vi "Main.vi"() -> ()   [LabVIEW 2020]
doc: "This template is for the Queued Message Handler design pattern.\n\nThe Event Handling Loop generates messages based on user interface actions.\n\nThe Message Handling Loop processes messages generated by the Event Handling Loop, or by other messages. The messages are string values, so new messages can be added easily to the Message Cases case structure in the Message Handling Loop. Each message cluster can also provide an optional value for Message Data, which is a variant that can be converted to whatever message-specific data is required."
uses:
  <vilib>/ErrorRing/Error Ring.xnode
  controls/oled UI Data.ctl
  support/Message Queue/oled Message Queue.lvlib
  support/User Event - Stop/oled User Event - Stop.lvlib
  support/Message Queue/Enqueue Message (Single).vi
  controls/HL Acq Data.ctl
  <vilib>/DAQmx/read.llb/DAQmx Read (Analog DBL 1Chan 1Samp).vi
  <vilib>/Instr/_visa.llb/VISA Configure Serial Port (Instr).vi
  <vilib>/DAQmx/create/channels.llb/DAQmx Create Channel (AI-Voltage-Basic).vi
  support/Message Queue/Enqueue Message (Array).vi
  controls/Acquisition data --typedef.ctl
  controls/Graph data --typedef.ctl
  <vilib>/Utility/error.llb/Error Cluster From Error Code.vi
  controls/Color --typedef.ctl
panel:
  in  "Color":T1 caption="Color de emisión"
  in  "Inicio de Barrido (V)":dbl
  out "Status":string
  in  "milliseconds to wait":i32=200
  out "Eff L-V":cluster{dbl[], dbl[]}(graph) caption="L-V"
  out "EFf I-V":cluster{dbl[], dbl[]}(graph) caption="L-V"
  in  "Puerto serial Fuente":refnum<visa-resource-name>="COM1"
  out "J-V":cluster{dbl[], dbl[]}(graph)
  out "L-V":cluster{dbl[], dbl[]}(graph)
  in  "OLED A":dbl=0.7 caption="Area del OLED [cm2]"
  in  "OLED-PD dist":dbl=1.0 caption="Distancia OLED-fotodiodo [cm]"
  in  "Protection C":dbl=0.1 caption="Corriente de Proteccion [A]\n(0.1-0.3A recomendado)"
  in  "Max V":dbl=10.0 caption="Voltaje máximo [V]\n(20V max. recomendado)"
  in  "Iniciar":bool
  in  "Step #":dbl=100.0 caption="Numero de pasos\n(100-250 recomendado)"
  in  "Exit":bool
  # "Sistema de caracterización de OLEDs"
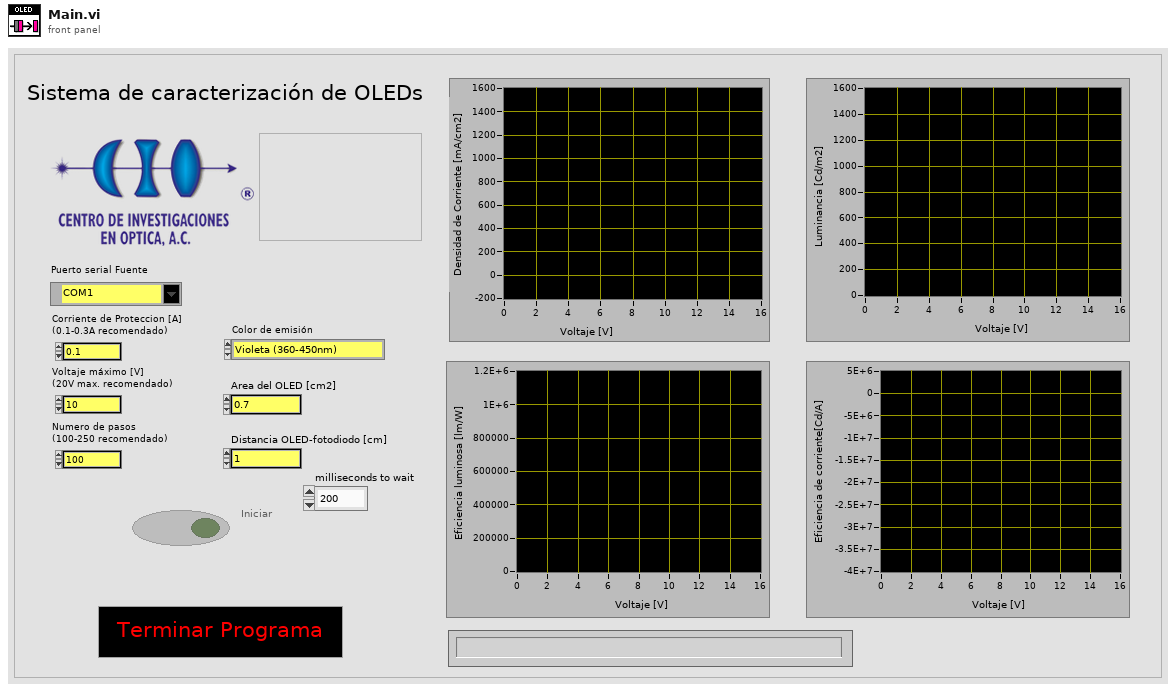
[diagram p1: front panel]
types:
  T1 = typedef "Color --typedef.ctl" = enum16{"Violeta (360-450nm)", "Azul (450-500nm)", "Verde(500-570nm)", "Amarillo (570-590nm)", "Naranja (600-610nm)", "Rojo (610-670nm)", "Blanco"}
  T2 = typedef "oled UI Data.ctl" = cluster{"Status":string, "Puerto serial":refnum<visa-resource-name>, "AI task":refnum<k21>, "Protection C":dbl, "Sweep start V":dbl, "Max V":dbl, "delta V":dbl, "Graph data":T3}
  T3 = typedef "Graph data --typedef.ctl" = cluster{"Voltaje [V]":dbl[], "Corriente [mA]":dbl[], "Densidad de corriente [CD/A]":dbl[], "Iluminancia [Lm/m2]":dbl[], "Luminance [Cd/m2]":dbl[], "Ef corriente [Cd/A]":dbl[], "Ef Luminosa [Cd/W]":dbl[], "V detector [V]":dbl[], "Pin [W]":dbl[]}
  T4 = cluster{"User event - Stop":refnum<user-event>, "User event - Sleep HL":refnum<user-event>, "User event -  Wake HL":refnum<user-event>}
  T5 = typedef "oled Message Queue.lvlib/All Message Queues.ctl" = cluster{"UI":refnum<queue>}
  T6 = enum8{"Enabled", "Disabled", "Disabled and Grayed Out"}
  T7 = typedef "HL Acq Data.ctl" = cluster{"dV":dbl, "Vmax":dbl, "Vo":dbl}
  T8 = typedef "Acquisition data --typedef.ctl" = cluster{"Iluminancia  lm/m2":dbl, "DAQ AV":dbl, "Luminancia (Cd/m2)":dbl, "Pin(W)":dbl, "SM V":dbl, "SM I":dbl, "OLED Area cm2":dbl}
  T9 = cluster{"Voltaje [V]":dbl[], "Luminance [Cd/m2]":dbl[]}
  T10 = cluster{"Voltaje [V]":dbl[], "V detector [V]":dbl[]}
  T11 = cluster{"Voltaje [V]":dbl[], "Ef corriente [Cd/A]":dbl[]}
  T12 = cluster{"Voltaje [V]":dbl[], "Corriente [mA]":dbl[]}
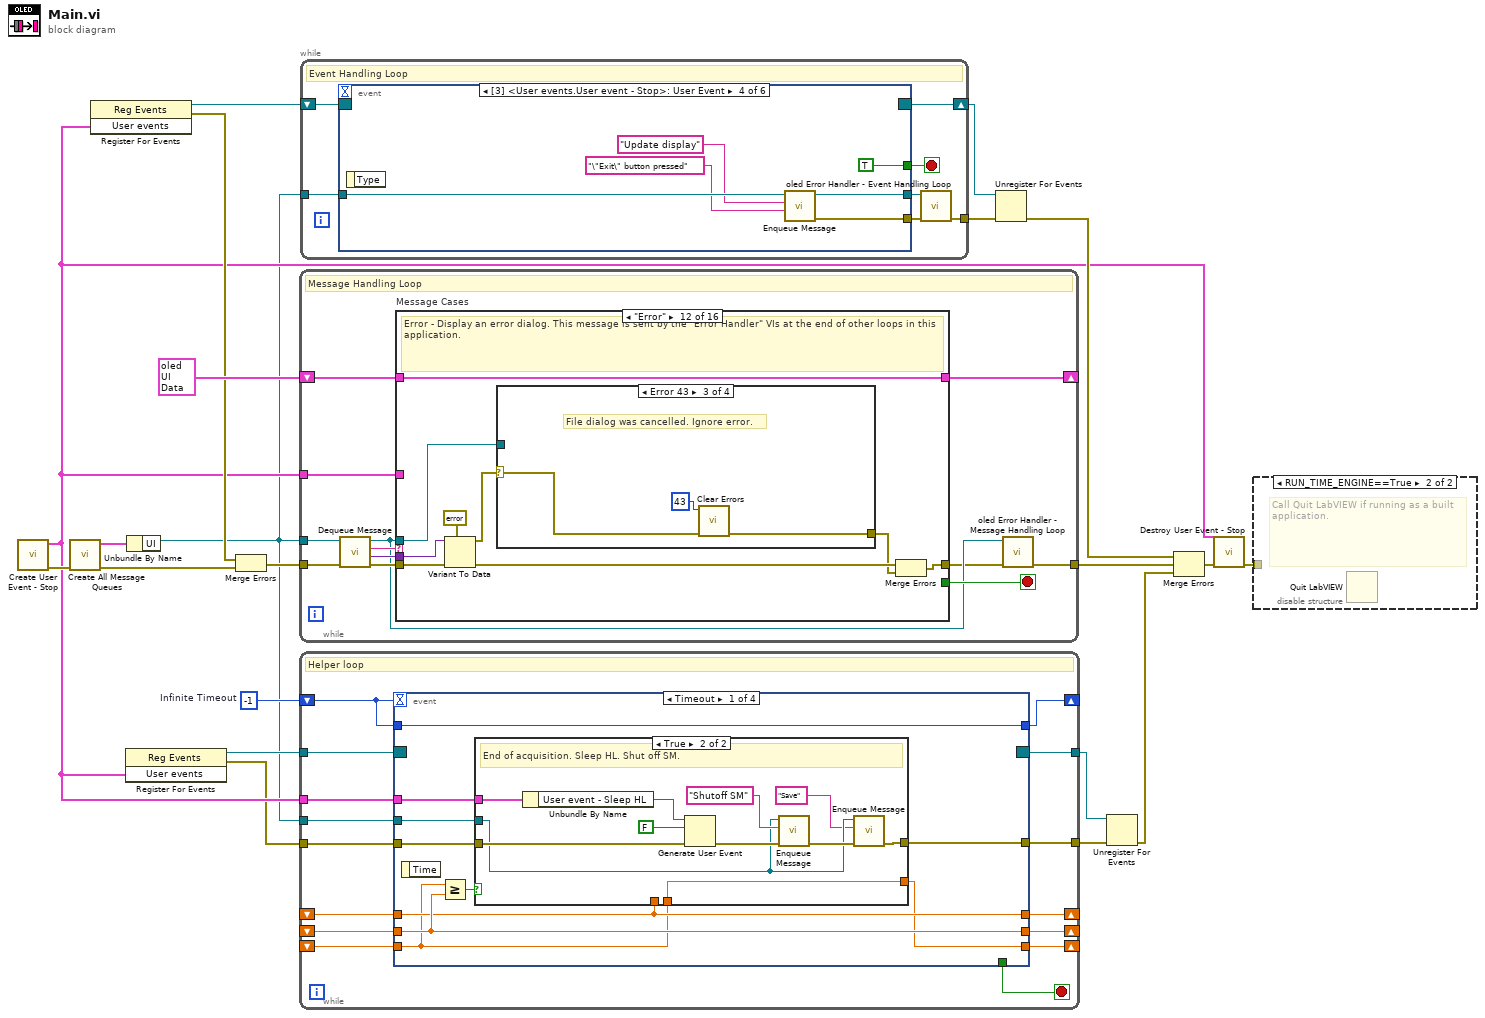
[diagram p0: block diagram]
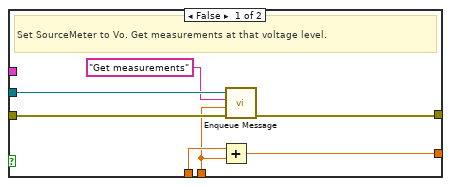
[diagram p2: hidden frame]
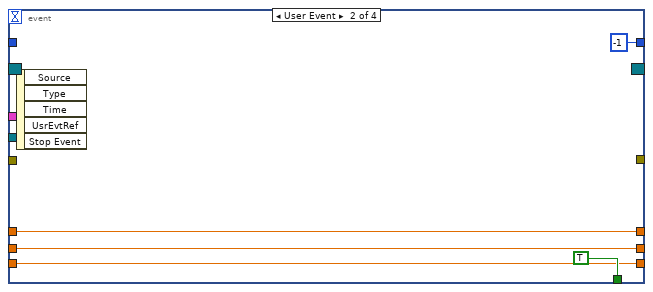
[diagram p3: hidden frame]
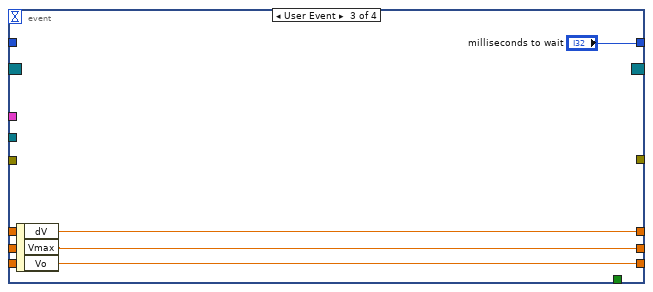
[diagram p4: hidden frame]
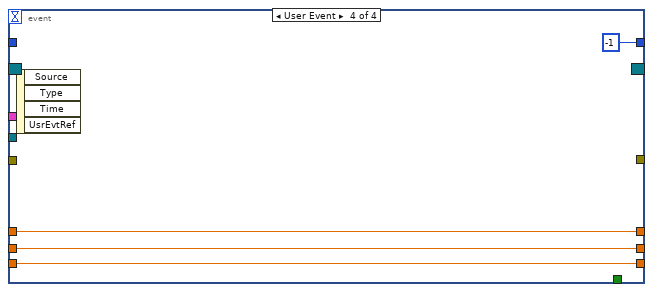
[diagram p5: hidden frame]
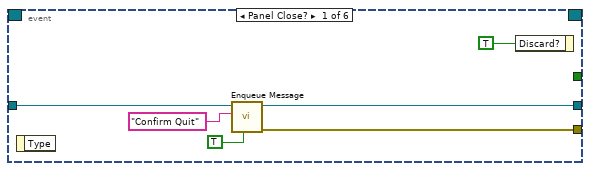
[diagram p6: hidden frame]
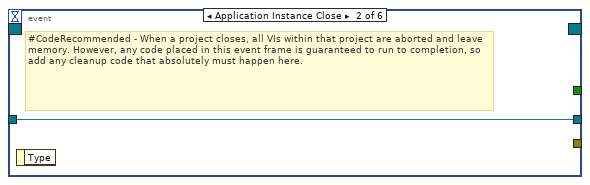
[diagram p7: hidden frame]
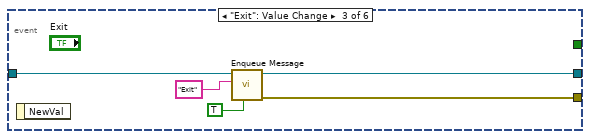
[diagram p8: hidden frame]
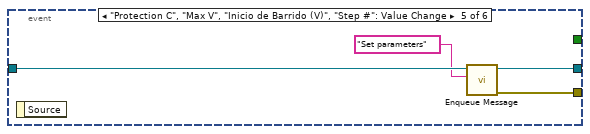
[diagram p9: hidden frame]
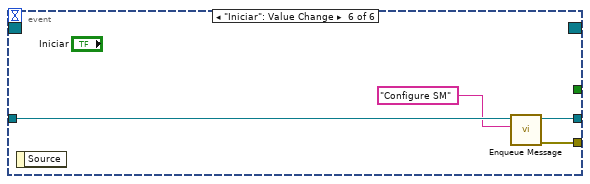
[diagram p10: hidden frame]
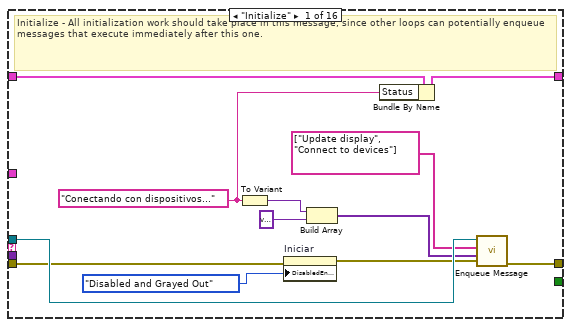
[diagram p11: hidden frame]
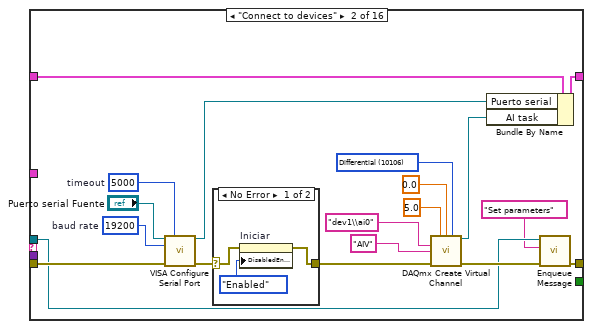
[diagram p12: hidden frame]
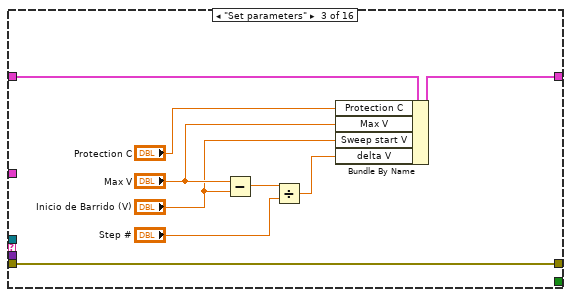
[diagram p14: hidden frame]
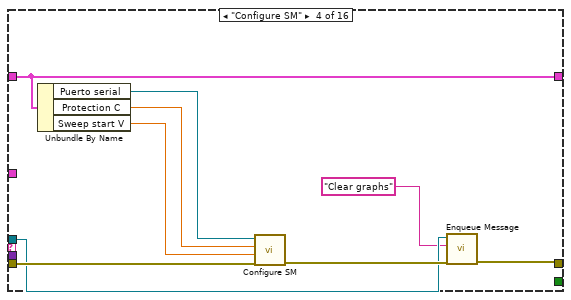
[diagram p15: hidden frame]
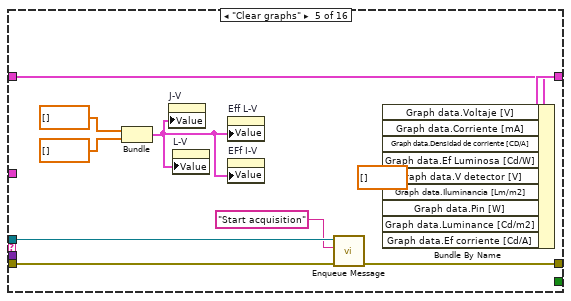
[diagram p16: hidden frame]
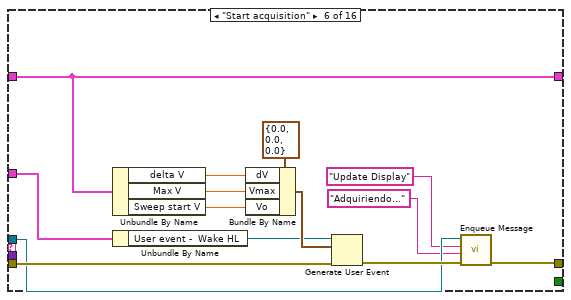
[diagram p17: hidden frame]
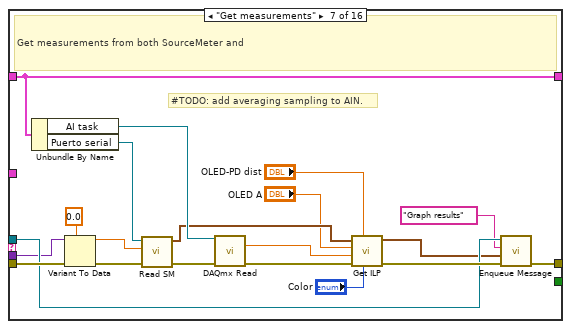
[diagram p18: hidden frame]
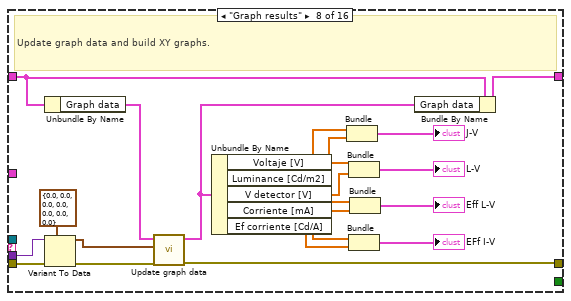
[diagram p19: hidden frame]
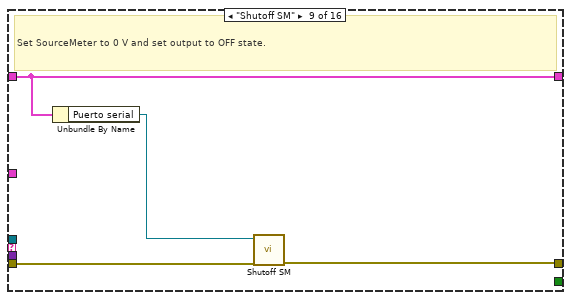
[diagram p20: hidden frame]
diagram:
  w9 = -1  # Infinite Timeout
  n1 = call "Create User Event - Stop.vi"() -> ("error out"=w19:errorcluster, "User events"=w4:T4)  [unwired: 10 in]
  n2 = call "Create All Message Queues.vi"("error in (no error)"=w19) -> ("error out"=w21:errorcluster, "Message Queues out"=w20:T5)  [unwired: 9 in]
  n3 = register-events(w4) -> (reference out=w12:refnum<event-registration>, error out=w10:errorcluster)  [unwired: 2 in]
  n4 = register-events(w4) -> (reference out=w8:refnum<event-registration>, error out=w2:errorcluster)  [unwired: 2 in]
  n5 = Unbundle By Name(w20) -> ("UI"=w1:refnum<queue>)
  n6 = Merge Errors(w10, w21) -> (w11:errorcluster)
  n7 = while {
    tunnel: w1 -> [w25]
    shift-right: [w32] -> _
    shift-left: T2 {"Status"="", "Puerto serial"="", "AI task"="", "Protection C"=0.0, "Sweep start V"=0.0, "Max V"=0.0, "delta V"=0.0, "Graph data"={"Voltaje [V]"=[], "Corriente [mA]"=[], "Densidad de corriente [CD/A]"=[], "Iluminancia [Lm/m2]"=[], "Luminance [Cd/m2]"=[], "Ef corriente [Cd/A]"=[], "Ef Luminosa [Cd/W]"=[], "V detector [V]"=[], "Pin [W]"=[]}} ("Data Cluster") -> [w33]
    tunnel: w4 -> [w30]
    tunnel: w11 -> [w29]
    tunnel: [w23] -> w6
    stop <- w31 stop-if-true
    # "Message Handling Loop"
    n8 = call "Dequeue Message.vi"("error in (no error)"=w29, "Message Queue"=w25) -> ("error out"=w28:errorcluster, "Message Data"=w26:variant, "Message"=w27:string, "dup Message Queue"=w24:refnum<queue>)  [unwired: 6 in]
    n9 = case "Message Cases" shown="\"Error\"" w27 {
      selector: w27 -> [_ _ _ _ _ _ _ _ _ _ _ _ _ _ _ w227]
      tunnel: w24 -> [w42 w49 _ w79 w88 w99 w122 _ _ _ _ w171 w196 _ w226 _]
      tunnel: w28 -> [w35 w64 w77 w82 w90 w105 w130 w149 w153 w155 w169 w179 w200 w203 w220 _]
      tunnel: [w45 w50 w77 w80 w89 w100 w123 w141 w152 w154 w170 w174 w198 w201 w223 w228] -> w22
      tunnel: w33 -> [w44 w60 w75 w86 w91 w103 w129 w144 w151 w157 w160 w178 w199 w202 w216 w229]
      tunnel: [w43 w58 w70 w86 w93 w103 w129 w143 w151 w157 w158 w178 w199 w202 w216 w229] -> w32
      tunnel: [_ _ _ _ _ _ _ _ _ _ _ _ _ _ TRUE _] -> w31
      tunnel: w26 -> [_ _ _ _ _ _ w113 w147 _ _ w168 w177 _ _ w217 _]
      tunnel: w30 -> [_ _ _ _ _ w106 _ _ _ _ _ _ _ _ w222 _]
      frame "Initialize" {
        w37 = "Conectando con dispositivos..." ("Initial Message")
        # "Initialize - All initialization work should take place in this message, since other loops can potentially enqueue messages that execute immediately after this one."
        n10 = To Variant(anything=w37) -> (Variant=w40:variant)
        n11 = property on="Iniciar" class="Bool (strict)"(error in=w35, "DisabledEnum"=T6."Disabled and Grayed Out" ("Disabled")) -> (error out=w34:errorcluster)  [unwired: 1 in, 1 out]
        n12 = Build Array(w40, variant ("element")) -> (w38:variant[])
        n13 = Bundle By Name(cluster=w44, "Status"=w37) -> (w43:T2)
        n14 = call-poly "Enqueue Message.vi"("error in (no error)"=w34, "Message Data Array"=w38, "Message Array"=string[] ["Update display", "Connect to devices"] ("Message"), "Message Queue"=w42) -> ("error out"=w45:errorcluster)  [unwired: 6 in, 1 out]
      }
      frame "Connect to devices" {
        w53 = 10106 items=["Default"=-1, "RSE"=10083, "NRSE"=10078, "Differential"=10106, "Pseudodifferential"=12529] ("input terminal configuration")
        w61 = u32 5000  # timeout
        w62 = u32 19200  # baud rate
        n15 = call-poly "VISA Configure Serial Port"("VISA resource name"="Puerto serial Fuente", "timeout (10sec)"=w61, "baud rate (9600)"=w62, "error in (no error)"=w64) -> ("VISA resource name out"=w59:refnum<visa-resource-name>, "error out"=w47:errorcluster)  [unwired: 3 in, 7 out]
        n16 = case shown="No Error" w47 {
          selector: w47 -> [w67 w68]
          tunnel: [w66 w68] -> w46
          frame No Error {
            n17 = property on="Iniciar" class="Bool (strict)"(error in=w67, "DisabledEnum"=T6."Enabled" ("Disabled")) -> (error out=w66:errorcluster)  [unwired: 1 in, 1 out]
          }
          frame Error {
          }
        }
        n18 = call-poly <vilib>:"DAQmx Create Virtual Channel.vi"("maximum value"=5.0, "minimum value"=0.0, "input terminal configuration"=w53, "physical channels"="dev1\\ai0", "name to assign"="AIV", "error in"=w46) -> ("task out"=w52:refnum<k21>, "error out"=w51:errorcluster)  [unwired: 8 in]
        n19 = Bundle By Name(cluster=w60, "Puerto serial"=w59, "AI task"=w52) -> (w58:T2)
        n20 = call-poly "Enqueue Message.vi"("error in (no error)"=w51, "Message"="Set parameters", "Message Queue"=w49) -> ("error out"=w50:errorcluster)  [unwired: 7 in, 1 out]
      }
      frame "Set parameters" {
        n21 = Subtract(x="Max V", y="Inicio de Barrido (V)") -> (x-y=w76:dbl)
        n22 = Divide(x=w76, y="Step #") -> (x/y=w71:dbl)
        n23 = Bundle By Name(cluster=w75, "Protection C"="Protection C", "Max V"="Max V", "Sweep start V"="Inicio de Barrido (V)", "delta V"=w71) -> (w70:T2)
      }
      frame "Configure SM" {
        n24 = Unbundle By Name(w86) -> ("Puerto serial"=w84:refnum<visa-resource-name>, "Protection C"=w83:dbl, "Sweep start V"=w85:dbl)
        n25 = call "Configure SM.vi"("error in (no error)"=w82, "Sweep start V"=w85, "Protection C"=w83, "Puerto serial"=w84) -> ("error out"=w81:errorcluster)  [unwired: 7 in]
        n26 = call-poly "Enqueue Message.vi"("error in (no error)"=w81, "Message"="Clear graphs", "Message Queue"=w79) -> ("error out"=w80:errorcluster)  [unwired: 7 in, 1 out]
      }
      frame "Clear graphs" {
        w92 = dbl[] []
        n27 = Bundle(dbl[] [], dbl[] []) -> (w94:cluster{dbl[], dbl[]})  [unwired: 1 out]
        n28 = property on="J-V" class="XYGraph (strict)"("Value"=w94) -> ()  [unwired: 2 in, 2 out]
        n29 = property on="L-V" class="XYGraph (strict)"("Value"=w94) -> ()  [unwired: 2 in, 2 out]
        n30 = property on="Eff L-V" class="XYGraph (strict)"("Value"=w94) -> ()  [unwired: 2 in, 2 out]
        n31 = property on="EFf I-V" class="XYGraph (strict)"("Value"=w94) -> ()  [unwired: 2 in, 2 out]
        n32 = call-poly "Enqueue Message.vi"("error in (no error)"=w90, "Message"="Start acquisition", "Message Queue"=w88) -> ("error out"=w89:errorcluster)  [unwired: 7 in, 1 out]
        n33 = Bundle By Name(cluster=w91, "Graph data.Voltaje [V]"=w92, "Graph data.Corriente [mA]"=w92, "Graph data.Densidad de corriente [CD/A]"=w92, "Graph data.Ef Luminosa [Cd/W]"=w92, "Graph data.V detector [V]"=w92, "Graph data.Iluminancia [Lm/m2]"=w92, "Graph data.Pin [W]"=w92, "Graph data.Luminance [Cd/m2]"=w92, "Graph data.Ef corriente [Cd/A]"=w92) -> (w93:T2)
      }
      frame "Start acquisition" {
        n34 = Unbundle By Name(w103) -> ("delta V"=w102:dbl, "Max V"=w108:dbl, "Sweep start V"=w107:dbl)
        n35 = Unbundle By Name(w106) -> ("User event -  Wake HL"=w104:refnum<user-event>)
        n36 = Bundle By Name(cluster=T7 {"dV"=0.0, "Vmax"=0.0, "Vo"=0.0} ("event data"), "dV"=w102, "Vmax"=w108, "Vo"=w107) -> (w109:T7)
        n37 = Generate User Event(user event=w104, event data cluster=w109, error in=w105) -> (error out=w101:errorcluster)  [unwired: 1 in, 1 out]
        n38 = call-poly "Enqueue Message.vi"("error in (no error)"=w101, "Message Data"="Adquiriendo..." ("Message"), "Message"="Update Display", "Message Queue"=w99) -> ("error out"=w100:errorcluster)  [unwired: 6 in, 1 out]
      }
      frame "Get measurements" {
        # "#TODO: add averaging sampling to AIN."
        # "Get measurements from both SourceMeter and"
        n39 = Unbundle By Name(w129) -> ("AI task"=w126:refnum<k21>, "Puerto serial"=w128:refnum<visa-resource-name>)
        n40 = Variant To Data(error in=w130, type=0.0, Variant=w113) -> (data=w112:dbl, error out=w115:errorcluster)
        n41 = call "Read SM.vi"("error in (no error)"=w115, "Vo"=w112, "Puerto serial"=w128) -> ("error out"=w127:errorcluster, "Acquistion Data"=w119:T8)  [unwired: 7 in]
        n42 = call-poly <vilib>:"DAQmx Read.vi"("task/channels in"=w126, "error in"=w127) -> ("data"=w118:dbl, "error out"=w125:errorcluster)  [unwired: 11 in, 1 out]
        n43 = call "Get ILP.vi"("Color"="Color", "OLED-PD dist"="OLED-PD dist", "error in (no error)"=w125, "DAQ V"=w118, "OLED A"="OLED A", "Acquistion Data"=w119) -> ("error out"=w124:errorcluster, "Acquistion Data"=w120:T8)  [unwired: 4 in]
        n44 = call-poly "Enqueue Message.vi"("error in (no error)"=w124, "Message Data"=w120, "Message"="Graph results", "Message Queue"=w122) -> ("error out"=w123:errorcluster)  [unwired: 6 in, 1 out]
      }
      frame "Graph results" {
        # "Update graph data and build XY graphs."
        n45 = Unbundle By Name(w144) -> ("Graph data"=w145:T3)
        n46 = Variant To Data(error in=w149, type=T8 {"Iluminancia  lm/m2"=0.0, "DAQ AV"=0.0, "Luminancia (Cd/m2)"=0.0, "Pin(W)"=0.0, "SM V"=0.0, "SM I"=0.0, "OLED Area cm2"=0.0} ("output cluster"), Variant=w147) -> (data=w146:T8, error out=w142:errorcluster)
        n47 = call "Update graph data.vi"("error in (no error)"=w142, "Acquisition data"=w146, "Graph data"=w145) -> ("error out"=w141:errorcluster, "Graph data"=w135:T3)  [unwired: 7 in]
        n48 = Unbundle By Name(w135) -> ("Voltaje [V]"=w134:dbl[], "Luminance [Cd/m2]"=w140:dbl[], "V detector [V]"=w133:dbl[], "Corriente [mA]"=w132:dbl[], "Ef corriente [Cd/A]"=w131:dbl[])
        n49 = Bundle("Voltaje [V]"=w134, "Luminance [Cd/m2]"=w140) -> (→"J-V":T9)  [unwired: 1 in]
        n50 = Bundle("Voltaje [V]"=w134, "V detector [V]"=w133) -> (→"L-V":T10)  [unwired: 1 in]
        n51 = Bundle("Voltaje [V]"=w134, "Ef corriente [Cd/A]"=w131) -> (→"EFf I-V":T11)  [unwired: 1 in]
        n52 = Bundle("Voltaje [V]"=w134, "Corriente [mA]"=w132) -> (→"Eff L-V":T12)  [unwired: 1 in]
        n53 = Bundle By Name(cluster=w144, "Graph data"=w135) -> (w143:T2)
      }
      frame "Shutoff SM" {
        # "Set SourceMeter to 0 V and set output to OFF state."
        n54 = Unbundle By Name(w151) -> ("Puerto serial"=w150:refnum<visa-resource-name>)
        n55 = call "Shutoff SM.vi"("error in (no error)"=w153, "Puerto serial"=w150) -> ("error out"=w152:errorcluster)  [unwired: 8 in, 1 out]
      }
      frame "Save" {
        n56 = Unbundle By Name(w157) -> ("Graph data"=w156:T3)
        n57 = call "Write file.vi"("error in (no error)"=w155, "Graph data"=w156) -> ("error out"=w154:errorcluster)  [unwired: 9 in]
      }
      frame "Update Display" {
        # "Update Display - Convert the message data to a string to display in the Data Display indicator."
        n58 = Variant To Data(error in=w169, type="", Variant=w168) -> (data=w164:string, error out=w162:errorcluster)
        n59 = Unbundle By Name(w160) -> ("Status"=w166:string)
        n60 = Format Into String(format string="\n%s", initial string=w166, error in=w162, w164) -> (resulting string=w159:string, error out=w161:errorcluster)
        n61 = property on="Status" class="Str"(error in=w161, "Value"=w159) -> (error out=w163:errorcluster)  [unwired: 1 in, 1 out]
        n62 = Bundle By Name(cluster=w160, "Status"=w159) -> (w158:T2)
        n63 = Merge Errors(w163) -> (w170:errorcluster)
      }
      frame "Error" {
        # "Error - Display an error dialog. This message is sent by the \"Error Handler\" VIs at the end of other loops in this application."
        n64 = Variant To Data(error in=w179, type=errorcluster {"status"=FALSE, "code"=0, "source"=""} ("error constant"), Variant=w177) -> (data=w173:errorcluster, error out=w175:errorcluster)
        n65 = case shown="Error 43" w173 {
          selector: w173 -> [_ w181 w186 w190]
          tunnel: [_ w180 w187 w193] -> w172
          tunnel: w171 -> [_ _ _ _]
          frame No Error {
          }
          frame Default {
            n66 = Unbundle By Name(w181) -> ("code"=w183:i32)
            n67 = call "oled Error logger.vi"("error in (no error)"=w181) -> ("error out"=w180:errorcluster)  [unwired: 10 in]
            n68 = Format Into String(format string="Error desconocido. Código de error: %d. ", w183) -> (resulting string=w182:string)  [unwired: 2 in, 1 out]
            n69 = One Button Dialog(message=w182) -> ()  [unwired: 1 in, 1 out]
          }
          frame Error {
            # "File dialog was cancelled. Ignore error."
            n70 = call <vilib>:"Clear Errors.vi"("error in (no error)"=w186, "specific error code to clear (0: all)"=43) -> ("error out"=w187:errorcluster)  [unwired: 4 in, 1 out]
          }
          frame Error {
            n71 = property on="Iniciar" class="Bool (strict)"(error in=w190, "DisabledEnum"=T6."Disabled and Grayed Out" ("Disabled")) -> (error out=w189:errorcluster)  [unwired: 1 in, 1 out]
            n72 = One Button Dialog(message="No se pudo conectar con el dispositivo VISA. Verifique la conexión física y los parámetros de comunicación.") -> ()  [unwired: 1 in, 1 out]
            n73 = call <vilib>:"Clear Errors.vi"("error in (no error)"=w189, "specific error code to clear (0: all)"=-1073807343) -> ("error out"=w193:errorcluster)  [unwired: 4 in, 1 out]
          }
        }
        n74 = Merge Errors(w175, w172) -> (w174:errorcluster)
      }
      frame "Confirm Quit" {
        # "#CodeNeeded - If you want to provide an \"Are you sure\" dialog (or some other notification) before the application exits, place that code here. This message is typically sent from a Panel Close? event."
        # "Confirm Quit - Message that can confirm whether or not the user wants to exit the application."
        n75 = call-poly "Enqueue Message.vi"("Priority Message? (F)"=TRUE, "error in (no error)"=w200, "Message"="Exit", "Message Queue"=w196) -> ("error out"=w197:errorcluster)  [unwired: 6 in, 1 out]
        n76 = Merge Errors(w197) -> (w198:errorcluster)
      }
      frame "---Copy This Frame---" {
        # "Duplicate this frame when creating new messages.  Change this comment in the duplicated frame to describe this message."
        n77 = Merge Errors(w203) -> (w201:errorcluster)
      }
      frame "Exit" {
        # "Stop the VI"
        # "Release the message queue reference"
        # "Close communicastion, stop AI task and exit application."
        n78 = Unbundle By Name(w216) -> ("Puerto serial"=w210:refnum<visa-resource-name>, "AI task"=w215:refnum<k21>)
        n79 = Variant To Data(type=errorcluster {"status"=FALSE, "code"=0, "source"=""} ("error constant"), Variant=w217) -> (data=w218:errorcluster)  [unwired: 1 in, 1 out]
        n80 = call <vilib>:"Simple Error Handler.vi"("error in (no error)"=w218) -> ()  [unwired: 4 in, 5 out]
        n81 = Unbundle By Name(w222) -> ("User event - Stop"=w208:refnum<user-event>)
        n82 = call "Shutoff SM.vi"("Puerto serial"=w210) -> ("error out"=w209:errorcluster, "Puerto serial"=w206:refnum<visa-resource-name>)  [unwired: 9 in]
        n83 = call <vilib>:"DAQmx Stop Task.vi"("task/channels in"=w215) -> ("task out"=w214:refnum<k21>, "error out"=w213:errorcluster)  [unwired: 13 in]
        n84 = Release Queue(queue=w226, error in (no error)=w220) -> (error out=w224:errorcluster)  [unwired: 1 in, 2 out]
        n85 = call <vilib>:"DAQmx Clear Task.vi"("task in"=w214, "error in"=w213) -> ("error out"=w211:errorcluster)  [unwired: 13 in]
        n86 = VISA Write(VISA resource name=w206, write buffer=":SYST:RSEN OFF\n" ("Comando"), error in (no error)=w209) -> (VISA resource name out=w205:refnum<visa-resource-name>, error out=w207:errorcluster)  [unwired: 1 out]
        n87 = VISA Close(VISA resource name=w205, error in (no error)=w207) -> (error out=w212:errorcluster)
        n88 = call "Fire User Event - Stop.vi"("User Event - Stop"=w208) -> ("error out"=w221:errorcluster)  [unwired: 10 in]
        n89 = Merge Errors(w221, w224, w212, w211) -> (w223:errorcluster)
      }
      frame Default {
        # "'Default' case only runs if there is a message that isn't defined in any of the other cases.  Output a programming error."
        n90 = xnode "Error Ring"("parameter 0"=w227) -> ("error out"=w228:errorcluster)
      }
    }
    n91 = call "oled Error Handler - Message Handling Loop.vi"("error in (no error)"=w22, "Message Queue"=w24) -> ("dup error in"=w23:errorcluster)  [unwired: 8 in, 1 out]
  }
  n92 = while {
    shift-right: [w249] -> _
    shift-left: w9 -> [w248]
    tunnel: w8 -> [w251]
    tunnel: [w247] -> w7
    shift-right: [w246] -> _
    shift-left: _ -> [w243]
    shift-right: [w245] -> _
    shift-left: _ -> [w242]
    shift-right: [w244] -> _
    shift-left: _ -> [w241]
    tunnel: w4 -> [w240]
    tunnel: [w239] -> w3
    tunnel: w2 -> [w238]
    tunnel: w1 -> [w237]
    stop <- w250 stop-if-true
    # "Helper loop"
    n93 = event shown="[0] Timeout" {
      selector: w251 -> [_ _ _ _]
      dyn-events: [_ _ _ _] -> w247
      timeout: w248 -> [_ _ _ _]
      tunnel: [_ TRUE _ _] -> w250
      tunnel: w248 -> [w261 _ _ _]
      tunnel: [w261 -1 ("Infinite Timeout") "milliseconds to wait" -1 ("Infinite Timeout")] -> w249
      tunnel: [w255 w282 w287 w291] -> w246
      tunnel: [w259 w281 w286 w290] -> w245
      tunnel: [w253 w280 w285 w289] -> w244
      tunnel: w243 -> [w255 w282 _ w291]
      tunnel: w242 -> [w259 w281 _ w290]
      tunnel: w241 -> [w254 w280 _ w289]
      tunnel: w240 -> [w258 _ _ _]
      tunnel: [w257 _ _ _] -> w239
      tunnel: w238 -> [w256 _ _ _]
      tunnel: w237 -> [w252 _ _ _]
      event Timeout {
        n94 = event-data() -> ()  [unwired: 1 in, 1 out]
        n95 = Greater Or Equal?(x=w254, y=w259) -> (x >= y?=w260:bool)
        n96 = case shown="True" w260 {
          tunnel: w258 -> [_ w279]
          tunnel: [w265 w271] -> w257
          tunnel: w256 -> [w266 w276]
          tunnel: w255 -> [w268 _]
          tunnel: w254 -> [w262 w275]
          tunnel: [w267 w275] -> w253
          tunnel: w252 -> [w264 w270]
          frame False {
            # "Set SourceMeter to Vo. Get measurements at that voltage level."
            n97 = Add(x=w268, y=w262) -> (x+y=w267:dbl)
            n98 = call-poly "Enqueue Message.vi"("error in (no error)"=w266, "Message Data"=w262, "Message"="Get measurements", "Message Queue"=w264) -> ("error out"=w265:errorcluster)  [unwired: 6 in, 1 out]
          }
          frame True {
            # "End of acquisition. Sleep HL. Shut off SM."
            n99 = Unbundle By Name(w279) -> ("User event - Sleep HL"=w278:refnum<user-event>)
            n100 = Generate User Event(user event=w278, event data cluster=FALSE ("event data"), error in=w276) -> (error out=w274:errorcluster)  [unwired: 1 in, 1 out]
            n101 = call-poly "Enqueue Message.vi"("error in (no error)"=w274, "Message"="Shutoff SM", "Message Queue"=w270) -> ("error out"=w272:errorcluster)  [unwired: 7 in, 1 out]
            n102 = call-poly "Enqueue Message.vi"("error in (no error)"=w272, "Message"="Save", "Message Queue"=w270) -> ("error out"=w271:errorcluster)  [unwired: 7 in, 1 out]
          }
        }
      }
      event User Event {
        n103 = event-data() -> ()  [unwired: 1 in, 5 out]
      }
      event User Event {
        n104 = event-data() -> ("dV"=w287:dbl, "Vmax"=w286:dbl, "Vo"=w285:dbl)  [unwired: 1 in]
      }
      event User Event {
        n105 = event-data() -> ()  [unwired: 1 in, 4 out]
      }
    }
  }
  n106 = while {
    tunnel: w1 -> [w299]
    shift-right: [w297] -> w16
    shift-left: w12 -> [w298]
    tunnel: [w293] -> w13
    stop <- w295 stop-if-true
    # "Event Handling Loop"
    n107 = event shown="[3] <User events.User event - Stop>: User Event" {
      selector: w298 -> [_ _ _ _ _ _]
      dyn-events: [_ _ _ _ _ _] -> w297
      timeout: _ -> [_ _ _ _ _ _]
      tunnel: [_ _ _ TRUE ("Discard?") _ _] -> w295
      tunnel: w299 -> [w304 w306 w311 w316 w321 w325]
      tunnel: [w303 _ w310 w314 w319 w323] -> w296
      tunnel: [w302 w306 w309 w315 w320 w324] -> w294
      event Panel Close? {
        n108 = event-data() -> ()  [unwired: 1 in, 1 out]
        n109 = call-poly "Enqueue Message.vi"("Priority Message? (F)"=TRUE, "Message"="Confirm Quit", "Message Queue"=w304) -> ("error out"=w303:errorcluster, "dup Message Queue"=w302:refnum<queue>)  [unwired: 7 in]
        n110 = event-data("Discard?"=TRUE) -> ()  [unwired: 1 in, 1 out]
      }
      event Application Instance Close {
        # "#CodeRecommended - When a project closes, all VIs within that project are aborted and leave memory. However, any code placed in this event frame is guaranteed to run to completion, so add any cleanup code that absolutely must happen here."
        n111 = event-data() -> ()  [unwired: 1 in, 1 out]
      }
      event "Exit": Value Change {
        n112 = event-data() -> ()  [unwired: 1 in, 1 out]
        n113 = call-poly "Enqueue Message.vi"("Priority Message? (F)"=TRUE, "Message"="Exit", "Message Queue"=w311) -> ("error out"=w310:errorcluster, "dup Message Queue"=w309:refnum<queue>)  [unwired: 7 in]
      }
      event User Event {
        n114 = event-data() -> ()  [unwired: 1 in, 1 out]
        n115 = call-poly "Enqueue Message.vi"("Message Data"="\"Exit\" button pressed" ("VI Stopped"), "Message"="Update display", "Message Queue"=w316) -> ("error out"=w314:errorcluster, "dup Message Queue"=w315:refnum<queue>)  [unwired: 7 in]
      }
      event "Protection C", "Max V", "Inicio de Barrido (V)", "Step #": Value Change {
        n116 = event-data() -> ()  [unwired: 1 in, 1 out]
        n117 = call-poly "Enqueue Message.vi"("Message"="Set parameters", "Message Queue"=w321) -> ("error out"=w319:errorcluster, "dup Message Queue"=w320:refnum<queue>)  [unwired: 8 in]
      }
      event "Iniciar": Value Change {
        n118 = event-data() -> ()  [unwired: 1 in, 1 out]
        n119 = call-poly "Enqueue Message.vi"("Message"="Configure SM", "Message Queue"=w325) -> ("error out"=w323:errorcluster, "dup Message Queue"=w324:refnum<queue>)  [unwired: 8 in]
      }
    }
    n120 = call "oled Error Handler - Event Handling Loop.vi"("error in (no error)"=w296, "Message Queue"=w294) -> ("dup error in"=w293:errorcluster)  [unwired: 8 in, 1 out]
  }
  n121 = Unregister For Events(event registration refnum=w16, error in=w13) -> (error out=w17:errorcluster)
  n122 = Unregister For Events(event registration refnum=w7, error in=w3) -> (error out=w5:errorcluster)
  n123 = Merge Errors(w17, w6, w5) -> (w18:errorcluster)
  n124 = call "Destroy User Event - Stop.vi"("error in (no error)"=w18, "User events"=w4) -> ("error out"=w14:errorcluster)  [unwired: 9 in]
  n125 = disable-structure shown="RUN_TIME_ENGINE==True" {
    disable-tunnel: w14 -> [_ _]
    frame condition #0 (active) {
    }
    frame condition #1 {
      # "Call Quit LabVIEW if running as a built application."
      n126 = Quit LabVIEW() -> ()  [unwired: 1 in]
    }
  }
